vi "FRC Test Team Number.vi"(7 "Team number":string) -> (8 "pass?":bool)   [LabVIEW 2027]
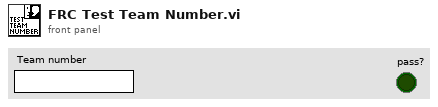
[diagram p1: front panel]
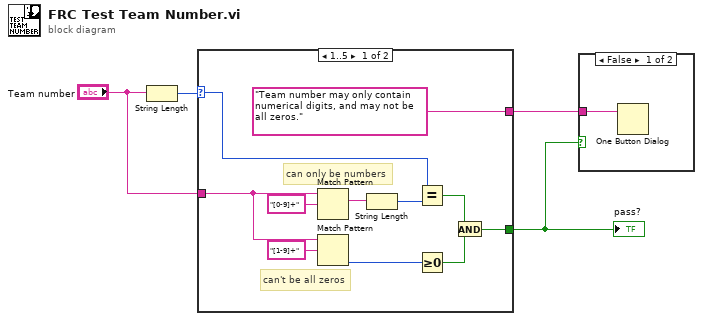
[diagram p0: block diagram]
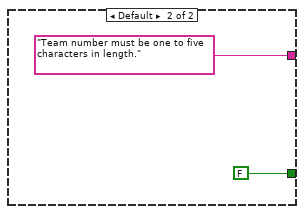
[diagram p3: hidden frame]
diagram:
  n1 = String Length(string="Team number") -> (length=w4:i32)
  n2 = case shown="1..5" w4 {
    selector: w4 -> [w7 _]
    tunnel: [w14 FALSE ("pass?")] -> w1
    tunnel: ["Team number may only contain numerical digits, and may not be all zeros." ("message") "Team number must be one to five characters in length." ("message")] -> w3
    tunnel: "Team number" -> [w11 _]
    frame 1..5 {
      # "can only be numbers"
      # "can't be all zeros"
      n3 = Match Pattern(string=w11, regular expression="[0-9]+") -> (match substring=w9:string)  [unwired: 1 in, 3 out]
      n4 = Match Pattern(string=w11, regular expression="[1-9]+") -> (offset past match=w10:i32)  [unwired: 1 in, 3 out]
      n5 = String Length(string=w9) -> (length=w8:i32)
      n6 = Equal?(x=w7, y=w8) -> (x = y?=w5:bool)
      n7 = Greater Or Equal To 0?(x=w10) -> (x >= 0?=w6:bool)
      n8 = And(x=w5, y=w6) -> (x .and. y?=w14:bool)
    }
    frame Default {
    }
  }
  "pass?" <- w1
  n9 = case shown="False" w1 {
    tunnel: w3 -> [w18 _]
    frame False {
      n10 = One Button Dialog(message=w18) -> ()  [unwired: 1 in, 1 out]
    }
    frame True {
    }
  }
